vi "CSMP-PostPostMsg.vi"(0 "State":string, 1 "Args":string, 2 "Source/target":string, 3 "Pre-State In":string, 4 "Pre-Args In":string, 5 "Error In":errorcluster caption="error in (no error)", 6 "Session Error":errorcluster, 8 "Module Name":string, 10 "Response Arguments":string) -> (14 "State Out":string, 15 "Args Out":string, 16 "Source/target Out":string, 17 "Pre-State Out":string, 18 "Pre-Args Out":string, 19 "Error":errorcluster)   [LabVIEW 2017, in "Communicable State Machine.lvlib"]
doc: "### CSMP-PostPostMsg.vi\n\n-- <b>Controls</b> --\n- <b>state</b>:\n- <b>args</b>:\n- <b>source/target</b>:\n- <b>Pre-State in</b>:\n- <b>Pre-Args in</b>:\n- <b>session error</b>:\n- <b>Module Name</b>:\n- <b>Response Arguments</b>:\n\n-- <b>Indicators</b> --\n- <b>state out</b>:\n- <b>args out</b>:\n- <b>source/target out</b>:\n- <b>Pre-State out</b>:\n- <b>Pre-Args out</b>:\n- <b>error</b>:"
uses:
  Communicable State Machine.lvlib
  Typedef/_Cross CSM State Data.ctl
  Typedef/_CSM_MSG_TYPE.ctl
  Typedef/_Cross CSM State Response.ctl
  Typedef/_CSM_Response Source Message.ctl
  Priority Queue/Enqueue Element.vi
  CSMQ/_CSMOFGV(lvlibp).vi
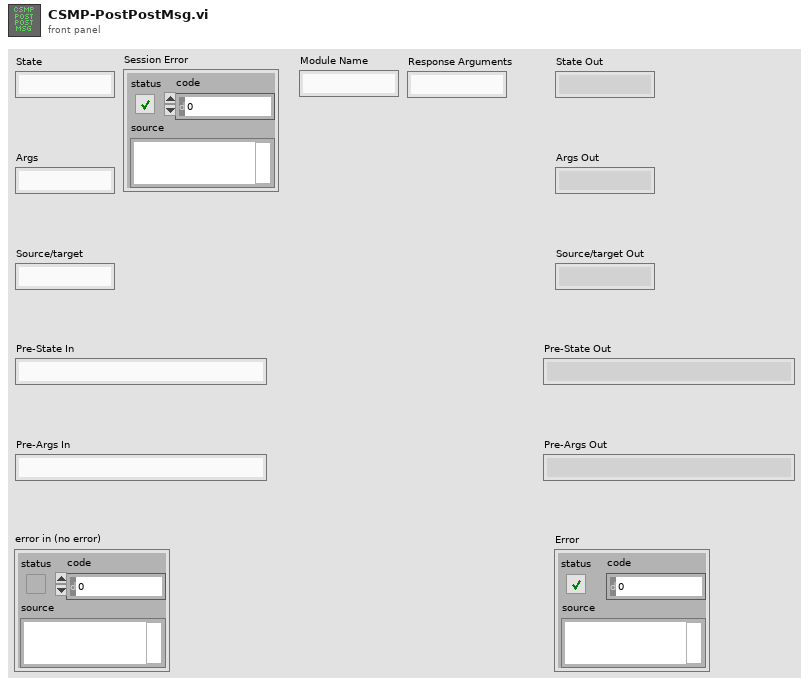
[diagram p1: front panel]
types:
  T1 = typedef "Communicable State Machine.lvlib/_CSM_MSG_TYPE.ctl" = enum16{"Sync Message(-@)", "Async Message(->)", "Async without Response(->|)", "Async Response", "Broadcast(-><all>)", "Broadcast(-><status>)", "Broadcast(-><interrupt>)", "Append to JKISM States", "Append to JKISM States(High Priority)", "Broadcast(-><state>)", "<None>"}
  T2 = typedef "Communicable State Machine.lvlib/_Cross CSM State Data.ctl" = cluster{"Msg Type":T1, "state":string, "args":string, "source":string, "RespQ":refnum<queue>, "Response For Message":T3, "Target":string}
  T3 = typedef "Communicable State Machine.lvlib/_CSM_Response Source Message.ctl" = cluster{"‘State":string, "’Arguments":string, "’Error":errorcluster}
  T4 = typedef "Communicable State Machine.lvlib/_CSMObj.ctl" = cluster{"info":T5, "Refs":T7}
  T5 = typedef "Communicable State Machine.lvlib/_CSMObj-Info.ctl" = cluster{"Module Name":string, "Requested Name":string, "Group Name":string, "Mode":T6, "Allowed Messages":string[]}
  T6 = typedef "Communicable State Machine.lvlib/_CSM_MODE.ctl" = enum16{"Not Exist", "Stand Alone", "CSM", "Worker", "Worker Agent", "Chain Node", "Chain"}
  T7 = typedef "Communicable State Machine.lvlib/_CSMObj-Refs.ctl" = cluster{"WatchDogQ":refnum<queue>, "CSMDataDVR":refnum<data-value>, "Queue":T8, "GroupDataDVR":refnum<data-value>, "TagMap":refnum<data-value>, "ExitEvent":refnum<user-event>, "NewStateEvent":refnum<user-event>, "StatusEvent":refnum<user-event>, "InterruptEvent":refnum<user-event>}
  T8 = typedef "Communicable State Machine.lvlib/Priority Queue.ctl" = cluster{"HPriorityQ":refnum<queue>, "LowPriorityQ":refnum<queue>}
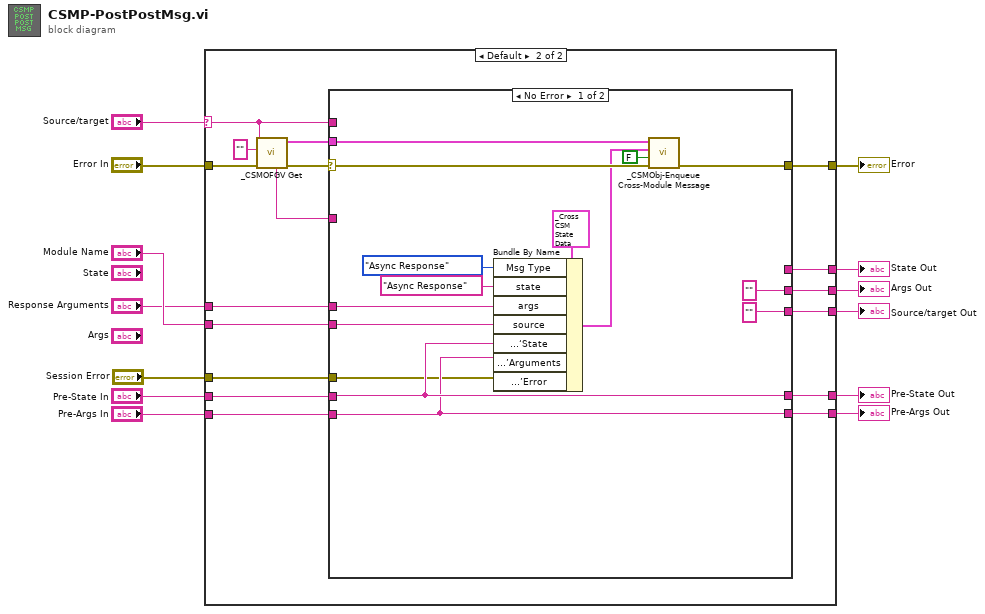
[diagram p0: block diagram]
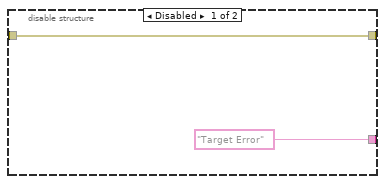
[diagram p4: hidden frame]
diagram:
  n1 = case shown="Default" "Source/target" {
    selector: "Source/target" -> [_ w29]
    tunnel: "Error In" -> [w14 w31]
    tunnel: [w14 w30] -> w12
    tunnel: [_ w28] -> w10
    tunnel: [_ w27] -> w9
    tunnel: "Pre-State In" -> [_ w26]
    tunnel: "Pre-Args In" -> [_ w25]
    tunnel: "Module Name" -> [_ w24]
    tunnel: "Response Arguments" -> [_ w23]
    tunnel: [_ w19] -> w4
    tunnel: [_ w18] -> w3
    tunnel: [_ w17] -> w2
    tunnel: "Session Error" -> [_ w16]
    frame "" {
    }
    frame Default {
      n2 = call "_CSMOFGV Get.vi"("Error In"=w31, "Message"="", "Name (\"\" to Use UUID) In"=w29) -> ("error out"=w21:errorcluster, "CSM-Obj"=w22:T4, "Name"=w20:string)  [unwired: 6 in]
      n3 = case shown="No Error" w21 {
        selector: w21 -> [w45 w47]
        tunnel: w22 -> [w46 _]
        tunnel: [_ w50] -> w19
        tunnel: w29 -> [_ w49]
        tunnel: w23 -> [w43 _]
        tunnel: w24 -> [w42 _]
        tunnel: w20 -> [_ _]
        tunnel: [w39 _] -> w28
        tunnel: w26 -> [w39 _]
        tunnel: w25 -> [w38 _]
        tunnel: [w38 _] -> w27
        tunnel: [w36 w48] -> w30
        tunnel: ["" ("Pre-State out") w49] -> w18
        tunnel: ["" ("Pre-Args out") w49] -> w17
        tunnel: w16 -> [w32 _]
        frame No Error {
          n4 = Bundle By Name(cluster=T2 {"Msg Type"=enum."Sync Message(-@)", "state"="", "args"="", "source"="", "RespQ"=refnum, "Response For Message"={"‘State"="", "’Arguments"="", "’Error"={"status"=FALSE, "code"=0, "source"=""}}, "Target"=""} ("Cross JKI State Machine State"), "Msg Type"=_CSM_MSG_TYPE."Async Response", "state"="Async Response" ("Response Arguments"), "args"=w43, "source"=w42, "Response For Message.‘State"=w39, "Response For Message.’Arguments"=w38, "Response For Message.’Error"=w32) -> (w41:T2)
          n5 = call "_CSMObj-Enqueue Cross-Module Message.vi"("Error In"=w45, "High Priority? (F)"=FALSE, "Data"=w41, "CSMQ In"=w46) -> ("error out"=w36:errorcluster)  [unwired: 6 in, 1 out]
        }
        frame Error {
          # "#github 242\nhttps://github.com/NEVSTOP-LAB/Communicable-State-Machine/issues/242\n\n异步的交互，有可能在没有完成前，返回的 target module 就退出了。\n通常这种情况不是bug 造成的，而是业务的逻辑，因此忽略掉这个 Target Error"
          n6 = disable-structure shown="Enabled" {
            disable-tunnel: ["Target Error" ("before match") _] -> w50
            disable-tunnel: [w51 _] -> w48
            disable-tunnel: w47 -> [w51 _]
            frame Disabled {
            }
            frame Enabled {
              # "#CSM-TODO\nthrow csm global event for this case"
            }
          }
        }
      }
    }
  }
  "State Out" <- w4
  "Args Out" <- w3
  "Source/target Out" <- w2
  "Error" <- w12
  "Pre-State Out" <- w10
  "Pre-Args Out" <- w9
